vi "Logic.vi"(8 "error in (no error)":errorcluster, 11 "CIFPlugin in":refnum<class "CAN_Writer_NIXNET_Plugin.lvclass">) -> (0 "error out":errorcluster, 3 "CIFPlugin out":refnum<class "CAN_Writer_NIXNET_Plugin.lvclass">)   [LabVIEW 2021, in "CAN_Writer_NIXNET_Plugin.lvclass"]
uses:
  CAN_Writer_NIXNET_Plugin.lvclass
  C:/Program Files/National Instruments/LabVIEW 2021/vi.lib/CIF Foundation/CIF Core/CIFCore/Class/CIFCorePlugin.lvclass
  <vilib>/CIF Foundation/CIF Core/CIFCore/Class/CIFCorePlugin.lvclass/CIFCorePlugin.ctl
  CAN_Writer_NIXNET_Plugin.lvclass/CAN_Writer_NIXNET_Plugin.ctl
  <vilib>/CIF Foundation/CIF CAN RW Core/CAN_RW_CORE.lvclass/CAN_RW_CORE.ctl
  Common/Typedef/Channels.ctl
  <vilib>/CIF Foundation/CIF Utilities/Statistics/I64/Stats_I64_CIF_U.lvclass/Stats_I64_CIF_U.ctl
  <vilib>/CIF Foundation/CIF Core/CIFCore/Common/Typedef/Multi_Cycle Logic State Enum.ctl
  <vilib>/CIF Foundation/CIF Core/CIFCore/Class/Accessors/Monitor/Write U64 1.vi
  <vilib>/CIF Foundation/CIF Core/CIFCore/Class/Accessors/Monitor/Write U64 2.vi
  <vilib>/CIF Foundation/CIF Core/CIFCore/Class/Accessors/Monitor/Write I64 1.vi
  <vilib>/CIF Foundation/CIF Core/CIFCore/Class/Accessors/Monitor/Write U64 3.vi
  <vilib>/CIF Foundation/CIF Core/CIFCore/Class/Accessors/Monitor/Write I64 2.vi
  <vilib>/CIF Foundation/CIF Core/CIFCore/Class/Benchmarking/Benchmark FIFO Read.vi
  <vilib>/CIF Foundation/CIF Core/CIFCore/Class/Accessors/Timestamps/Write Execute TS.vi
  <vilib>/CIF Foundation/CIF Core/CIFCore/Class/Accessors/Timestamps/Write Target Wake TS.vi
  <vilib>/CIF Foundation/CIF Utilities/Time/System Time/Get System Time.vi
  <vilib>/CIF Foundation/CIF Core/CIFCore/Class/Utilities/Clocks/External Clock to System Clock.vi
  <vilib>/CIF Foundation/CIF Core/CIFCore/Class/Benchmarking/Timestamp T_Out Control.vi
  <vilib>/CIF Foundation/CIF Utilities/Statistics/I64/X1 minus X0.vi
  <vilib>/CIF Foundation/CIF Utilities/Statistics/I64/Cyclic.vi
  <vilib>/CIF Foundation/CIF Core/CIFCore/Class/Benchmarking/Reset Delay.vi
  <vilib>/CIF Foundation/CIF Core/CIFCore/Class/Accessors/Timestamps/Write Sleep TS.vi
  <vilib>/CIF Foundation/CIF Core/CIFCore/Class/Accessors/Timestamps/Read Execute TS.vi
  <vilib>/CIF Foundation/CIF Core/CIFCore/Class/Accessors/Timestamps/Read Sleep TS.vi
  <vilib>/CIF Foundation/CIF Core/CIFCore/Class/Accessors/Timestamps/Read Target Wake TS.vi
  <vilib>/CIF Foundation/CIF CAN RW Core/Utilities/Reset Statistics.vi
  <vilib>/CIF Foundation/CIF CAN RW Core/Accessors/Read Statistcs.vi
  <vilib>/CIF Foundation/CIF Core/CIFCore/Class/Accessors/Read Refresh.vi
  <vilib>/CIF Foundation/CIF Utilities/Time/External Clocks/External Time to System Time.vi
  <vilib>/CIF Foundation/CIF Core/CIFCore/Class/Benchmarking/Benchmark FIFO Output.vi
  <vilib>/CIF Foundation/CIF Utilities/Statistics/I64/X1 minus X0.vi/dfabcf33-0dbc-4041-80a5-3dc0c86d2989.vi
  <vilib>/CIF Foundation/CIF Utilities/Statistics/I64/Cyclic.vi/dfabcf33-0dbc-4041-80a5-3dc0c86d2989.vi
  <vilib>/CIF Foundation/CIF Utilities/Time/SubVIs/Add Error.vi
  <vilib>/CIF Foundation/CIF Utilities/Statistics/I64/X1 minus X0.vi/dfabcf33-0dbc-4041-80a5-3dc0c86d2989.vi/9eb60a9a-770f-4d2d-8b3f-8465c267ecc9.vi
  <vilib>/CIF Foundation/CIF Utilities/Statistics/I64/Cyclic.vi/dfabcf33-0dbc-4041-80a5-3dc0c86d2989.vi/9eb60a9a-770f-4d2d-8b3f-8465c267ecc9.vi
  <vilib>/CIF Foundation/CIF XNET CAN RW/XNET CAN RW.lvclass
  C:/Program Files/National Instruments/LabVIEW 2021/vi.lib/CIF Foundation/CIF CAN RW Core/CAN_RW_CORE.lvclass
  <vilib>/CIF Foundation/CIF Utilities/Time/SubVIs/Error Core.vi
  <vilib>/CIF Foundation/CIF Utilities/Time/System Time/Sleep Until Future Time.vi
  <vilib>/CIF Foundation/CIF Channels Core/CIFChannels/CIFChannels.lvclass
  Common/CAN_Writer_NIXNET_Common.lvlib
  <vilib>/CIF Foundation/CIF Core/CIFCore/Class/CIFCorePlugin.lvclass
  <vilib>/CIF Foundation/CIF Core/CIFCore/Common/CIFCoreCommon.lvlib
  D:/dev/Plugins/CAN_Writer_NIXNET/Class/CAN_Writer_NIXNET_Plugin.lvclass
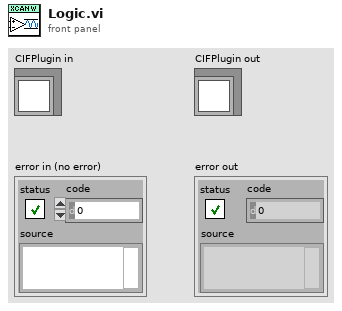
[diagram p1: front panel]
types:
  T1 = typedef "CAN_Writer_NIXNET_Common.lvlib/Channels.ctl" = enum16{"CAN_Frames"}
  T2 = typedef "CIFCoreCommon.lvlib/Multi_Cycle Logic State Enum.ctl" = enum16{"Read FIFO", "Sleep", "Output Data"}
  T3 = typedef "ChannelCommon.lvlib/FIFO Header.ctl" = cluster{"Length":u64, "T0":i64, "T_Out":i64, "T_Tx":i64, "Ctr":u64, "ClockID":u8}
  T4 = typedef "CIFCoreCommon.lvlib/FIFO Drop Internal Data.ctl" = cluster{"Last FIFO Ctr":u64, "FIFO Ctr Valid":bool}
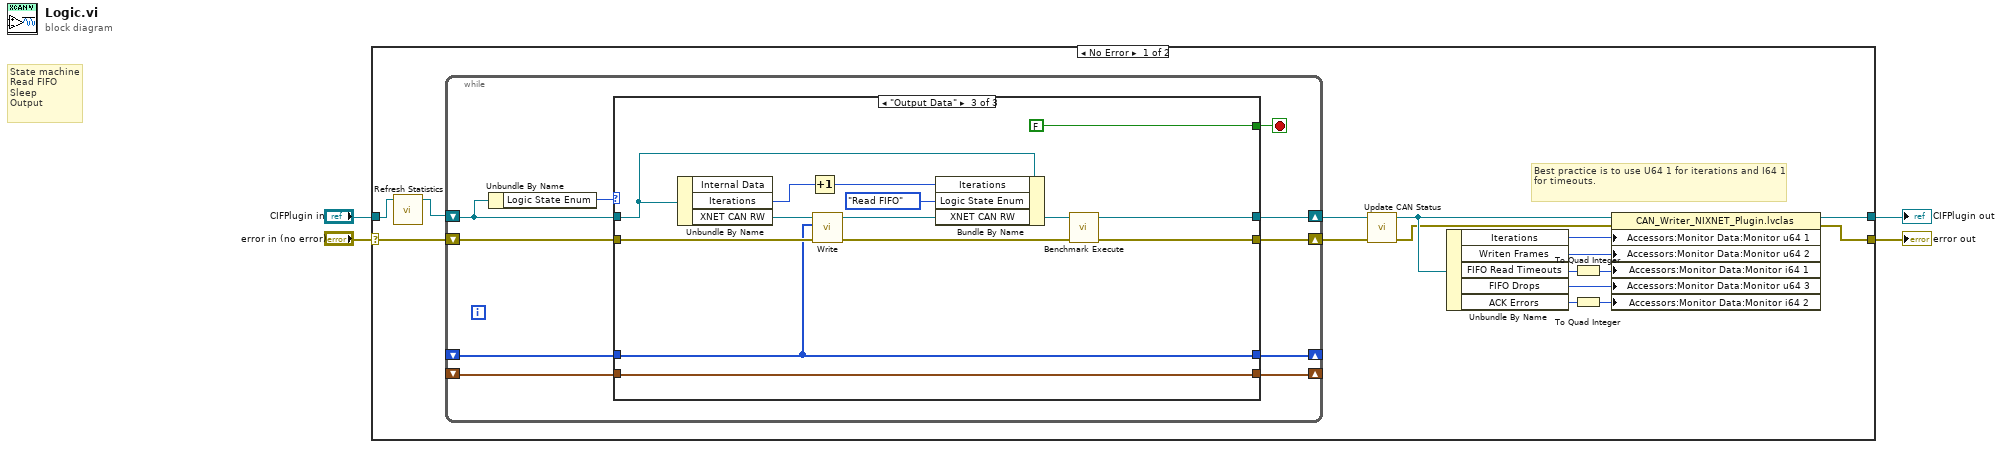
[diagram p0: block diagram]
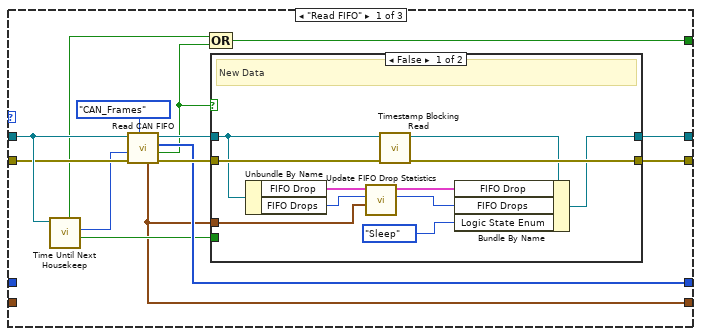
[diagram p2: hidden frame]
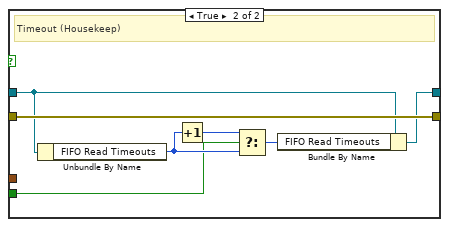
[diagram p3: hidden frame]
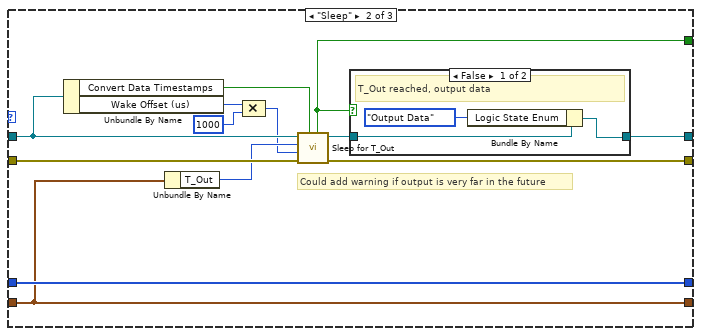
[diagram p4: hidden frame]
diagram:
  # "State machine\nRead FIFO\nSleep\nOutput"
  n1 = case shown="No Error" "error in (no error)" {
    selector: "error in (no error)" -> [w20 w95]
    tunnel: [w14 w95] -> w2
    tunnel: [w15 w94] -> w1
    tunnel: "CIFPlugin in" -> [w19 w94]
    frame No Error {
      # "Best practice is to use U64 1 for iterations and I64 1 for timeouts."
      n2 = call "Refresh Statistics.vi"("CIFPlugin in"=w19) -> ("CIFPlugin out"=w18:refnum<class "CAN_Writer_NIXNET_Plugin.lvclass">)  [unwired: 10 in]
      n3 = while {
        shift-right: [w29] -> w6
        shift-left: w18 -> [w24]
        shift-right: [w30] -> w7
        shift-left: w20 -> [w28]
        shift-right: [w26] -> _
        shift-left: _ -> [w22]
        shift-right: [w25] -> _
        shift-left: _ -> [w21]
        stop <- w27 stop-if-true
        n4 = Unbundle By Name(w24) -> ("Logic State Enum"=w23:T2)
        n5 = case shown="\"Output Data\"" w23 {
          tunnel: [w44 w71 w89] -> w30
          tunnel: [w43 w66 w88] -> w29
          tunnel: w24 -> [w42 w73 w91]
          tunnel: w28 -> [w41 w75 w92]
          tunnel: [w33 w68 FALSE ("Timeout (Housekeep now)")] -> w27
          tunnel: [w36 w70 w90] -> w26
          tunnel: [w31 w69 w86] -> w25
          tunnel: w22 -> [_ w70 w90]
          tunnel: w21 -> [_ w69 w86]
          frame "Read FIFO" {
            n6 = call <vilib>:"Time Until Next Housekeep.vi"("CIFCorePlugin in"=w42) -> ("Timeout Valid"=w32:bool, "Time Until Next Housekeep (ms)"=w39:i32, "Housekeep Now"=w35:bool)  [unwired: 7 in, 1 out]
            n7 = call <vilib>:"Read CAN FIFO.vi"("Channel Index"=Channels."CAN_Frames" ("Channels"), "error in (no error)"=w41, "Timeout (ms)"=w39, "CIFCorePlugin in"=w42) -> ("error out"=w37:errorcluster, "timed out?"=w34:bool, "Data"=w36:u8[], "CIFCorePlugin out"=w38:refnum<class "CAN_Writer_NIXNET_Plugin.lvclass">, "Header"=w31:T3)  [unwired: 3 in]
            n8 = Compound Arithmetic op=OR(w35, w34) -> (w33:bool)
            n9 = case shown="False" w34 {
              tunnel: w38 -> [w51 w57]
              tunnel: w37 -> [w55 w62]
              tunnel: [w52 w58] -> w43
              tunnel: [w54 w62] -> w44
              tunnel: w32 -> [_ w56]
              tunnel: w31 -> [w48 _]
              frame False {
                # "New Data"
                n10 = Unbundle By Name(w51) -> ("FIFO Drop"=w49:T4, "FIFO Drops"=w45:u64)
                n11 = call <vilib>:"Update FIFO Drop Statistics.vi"("Header"=w48, "FIFO Drop Stat in"=w45, "FIFO Drop in"=w49) -> ("FIFO Drops Stat out"=w46:u64, "FIFO Drop out"=w47:T4)  [unwired: 7 in]
                n12 = call <vilib>:"Timestamp Blocking Read.vi"("error in (no error)"=w55, "CIFCorePlugin in"=w51) -> ("error out"=w54:errorcluster, "CIFCorePlugin out"=w53:refnum<class "CAN_Writer_NIXNET_Plugin.lvclass">)  [unwired: 8 in]
                n13 = Bundle By Name(cluster=w53, "FIFO Drop"=w47, "FIFO Drops"=w46, "Logic State Enum"=Multi_Cycle_Logic_State_Enum."Sleep") -> (w52:refnum<class "CAN_Writer_NIXNET_Plugin.lvclass">)
              }
              frame True {
                # "Timeout (Housekeep)"
                n14 = Unbundle By Name(w57) -> ("FIFO Read Timeouts"=w59:u64)
                n15 = Increment(x=w59) -> (x+1=w60:u64)
                n16 = Select(t=w60, s=w56, f=w59) -> (s? t:f=w61:u64)
                n17 = Bundle By Name(cluster=w57, "FIFO Read Timeouts"=w61) -> (w58:refnum<class "CAN_Writer_NIXNET_Plugin.lvclass">)
              }
            }
          }
          frame "Sleep" {
            # "Could add warning if output is very far in the future"
            n18 = Unbundle By Name(w73) -> ("Convert Data Timestamps"=w72:bool, "Wake Offset (us)"=w65:i64)
            n19 = Unbundle By Name(w69) -> ("T_Out"=w74:i64)
            n20 = Compound Arithmetic op=MULTIPLY(w65, i64 1000 ("value")) -> (w63:i64)
            n21 = call <vilib>:"Sleep for T_Out.vi"("Convert External Clocks (T)"=w72, "error in (no error)"=w75, "Wake Offset (2000 ns)"=w63, "T_Out (ns)"=w74, "CIFCorePlugin in"=w73) -> ("error out"=w71:errorcluster, "CIFCorePlugin out"=w67:refnum<class "CAN_Writer_NIXNET_Plugin.lvclass">, "Timeout (Housekeep now)"=w68:bool)  [unwired: 3 in, 1 out]
            n22 = case shown="False" w68 {
              tunnel: w67 -> [w77 w79]
              tunnel: [w76 w79] -> w66
              frame False {
                # "T_Out reached, output data"
                n23 = Bundle By Name(cluster=w77, "Logic State Enum"=Multi_Cycle_Logic_State_Enum."Output Data") -> (w76:refnum<class "CAN_Writer_NIXNET_Plugin.lvclass">)
              }
              frame True {
                # "No T-Out, housekeep"
              }
            }
          }
          frame "Output Data" {
            n24 = Unbundle By Name(w91) -> ("Iterations"=w80:u64, "XNET CAN RW"=w93:refnum<class "XNET CAN RW.lvclass">)  [unwired: 1 out]
            n25 = Increment(x=w80) -> (x+1=w81:u64)
            n26 = call-dynamic "Write.vi"("error in (no error)"=w92, "pcap CAN DATA in"=w90, "XNET_CAN_RW in"=w93) -> ("error out"=w82:errorcluster, "XNET_CAN_RW out"=w84:refnum<class "XNET CAN RW.lvclass">)  [unwired: 6 in, 1 out]
            n27 = Bundle By Name(cluster=w91, "Iterations"=w81, "Logic State Enum"=Multi_Cycle_Logic_State_Enum."Read FIFO", "XNET CAN RW"=w84) -> (w83:refnum<class "CAN_Writer_NIXNET_Plugin.lvclass">)
            n28 = call <vilib>:"Benchmark Execute.vi"("error in (no error)"=w82, "CIFCorePlugin in"=w83) -> ("error out"=w89:errorcluster, "CIFCorePlugin out"=w88:refnum<class "CAN_Writer_NIXNET_Plugin.lvclass">)  [unwired: 8 in]
          }
        }
      }
      n29 = call "Update CAN Status.vi"("error in (no error)"=w7, "CAN_Writer_NIXNET_Plugin in"=w6) -> ("error out"=w5:errorcluster, "CAN_Writer_NIXNET_Plugin out"=w8:refnum<class "CAN_Writer_NIXNET_Plugin.lvclass">)  [unwired: 8 in]
      n30 = Unbundle By Name(w8) -> ("Iterations"=w17:u64, "Writen Frames"=w16:u64, "FIFO Read Timeouts"=w13:u64, "FIFO Drops"=w11:u64, "ACK Errors"=w10:u64)
      n31 = To Quad Integer(1:w13) -> (0:w12:i64)
      n32 = To Quad Integer(1:w10) -> (0:w9:i64)
      n33 = property class="CAN_Writer_NIXNET_Plugin.lvclas"(reference=w8, error in=w5, "Accessors:Monitor Data:Monitor u64 1"=w17, "Accessors:Monitor Data:Monitor u64 2"=w16, "Accessors:Monitor Data:Monitor i64 1"=w12, "Accessors:Monitor Data:Monitor u64 3"=w11, "Accessors:Monitor Data:Monitor i64 2"=w9) -> (reference out=w15:refnum<class "CAN_Writer_NIXNET_Plugin.lvclass">, error out=w14:errorcluster)
    }
    frame Error {
    }
  }
  "error out" <- w2
  "CIFPlugin out" <- w1
